vi "set OBW Limit Frequency.vi"(8 "error in (no error)":errorcluster, 9 "Limit On?":bool, 10 "Limit Frequency (Hz)":dbl format="%#_6p", 11 "Keysight 9020A in":refnum<class "Keysight 9020A.lvclass">) -> (0 "error out":errorcluster, 3 "Keysight 9020A out":refnum<class "Keysight 9020A.lvclass">)   [LabVIEW 2023, in "Spectrum Analyzer.lvlib" / "Keysight 9020A.lvclass"]
uses:
  Keysight 9020A.lvclass
  Keysight 9020A.lvclass/Keysight 9020A.ctl
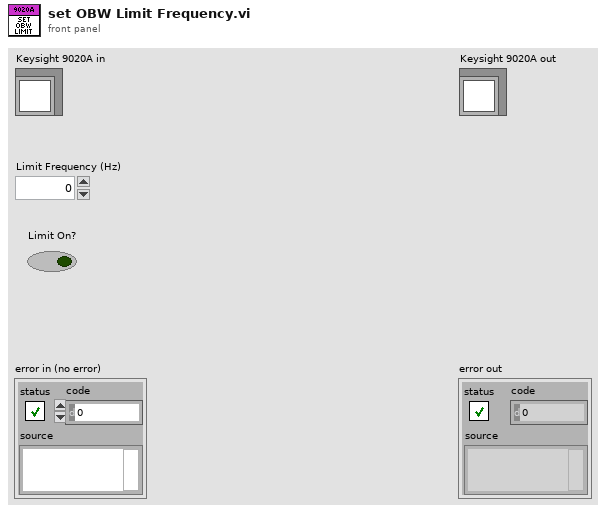
[diagram p1: front panel]
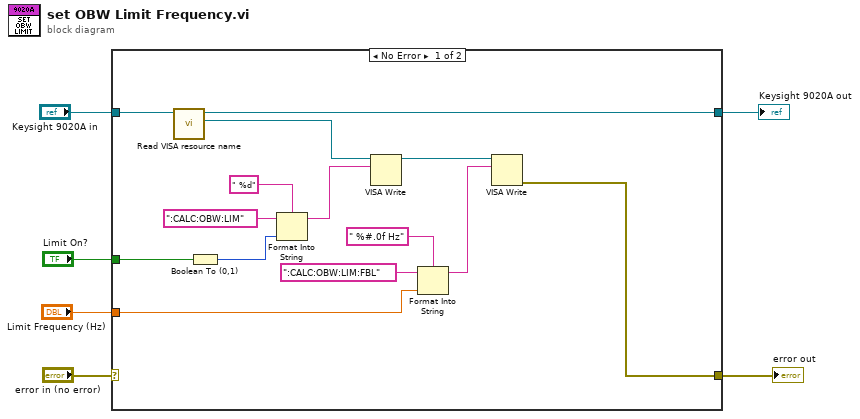
[diagram p0: block diagram]
diagram:
  n1 = case shown="No Error" "error in (no error)" {
    selector: "error in (no error)" -> [_ w21]
    tunnel: "Keysight 9020A in" -> [w20 w22]
    tunnel: [w19 w22] -> w5
    tunnel: [w7 w21] -> w3
    tunnel: "Limit On?" -> [w14 _]
    tunnel: "Limit Frequency (Hz)" -> [w9 _]
    frame No Error {
      n2 = call "Read VISA resource name.vi"("Keysight 9020A in"=w20) -> ("VISA resource name"=w17:refnum<visa-resource-name>, "Keysight 9020A out"=w19:refnum<class "Keysight 9020A.lvclass">)  [unwired: 8 in, 1 out]
      n3 = Boolean To (0,1)(Boolean=w14) -> (0, 1=w13:i16)
      n4 = Format Into String(format string=" %d", initial string=":CALC:OBW:LIM" ("string"), w13) -> (resulting string=w16:string)  [unwired: 1 in, 1 out]
      n5 = VISA Write(VISA resource name=w17, write buffer=w16) -> (VISA resource name out=w12:refnum<visa-resource-name>)  [unwired: 1 in, 2 out]
      n6 = Format Into String(format string=" %#.0f Hz", initial string=":CALC:OBW:LIM:FBL" ("write buffer"), w9) -> (resulting string=w8:string)  [unwired: 1 in, 1 out]
      n7 = VISA Write(VISA resource name=w12, write buffer=w8) -> (error out=w7:errorcluster)  [unwired: 1 in, 2 out]
    }
    frame Error {
    }
  }
  "error out" <- w3
  "Keysight 9020A out" <- w5
